vi "Requests from uServices.vi"(8 "error in (no error)":errorcluster, 9 "Data":variant, 10 "Requests":T1, 11 "Guardian in":refnum<class "Guardian.lvclass">) -> (0 "error out":errorcluster, 3 "Guardian out":refnum<class "Guardian.lvclass">)   [LabVIEW 2020, in "TALOS.lvlib" / "Guardian.lvlib" / "Guardian.lvclass"]
uses:
  Guardian.lvclass
  Guardian Messages/Broadcast to Guardians Msg/Broadcast to Guardians Msg.lvclass
  builds/Actor Framework PPL/Actor Framework.lvlibp/1abvi3w/vi.lib/ActorFramework/Actor/Actor.lvclass
  TALOS.lvlib
  Guardian Messages/Message to uService Msg/Message to uService Msg.lvclass
  C:/LabVIEW Code/TALOS/talos/Ancestor/Ancestor/Ancestor.lvclass
  C:/LabVIEW Code/TALOS/builds/Actor Framework PPL/Actor Framework.lvlibp/1abvi3w/vi.lib/ActorFramework/Actor/Actor.lvclass
  C:/LabVIEW Code/TALOS/talos/Guardian/Guardian/Guardian.lvclass
  Requests.ctl
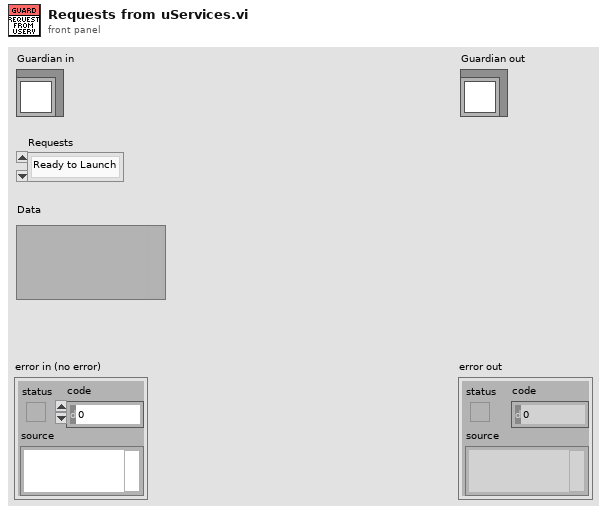
[diagram p1: front panel]
types:
  T1 = typedef "TALOS.lvlib/Guardian.lvlib/Guardian.lvclass/Requests.ctl" = enum16{"Ready to Launch", "Start RUN", "Stop RUN", "Update DAQ Params", "Update Error Listbox", "Update Run Status", "Update Kasli Log", "Run Stopped with Errors", "Switch uS View"}
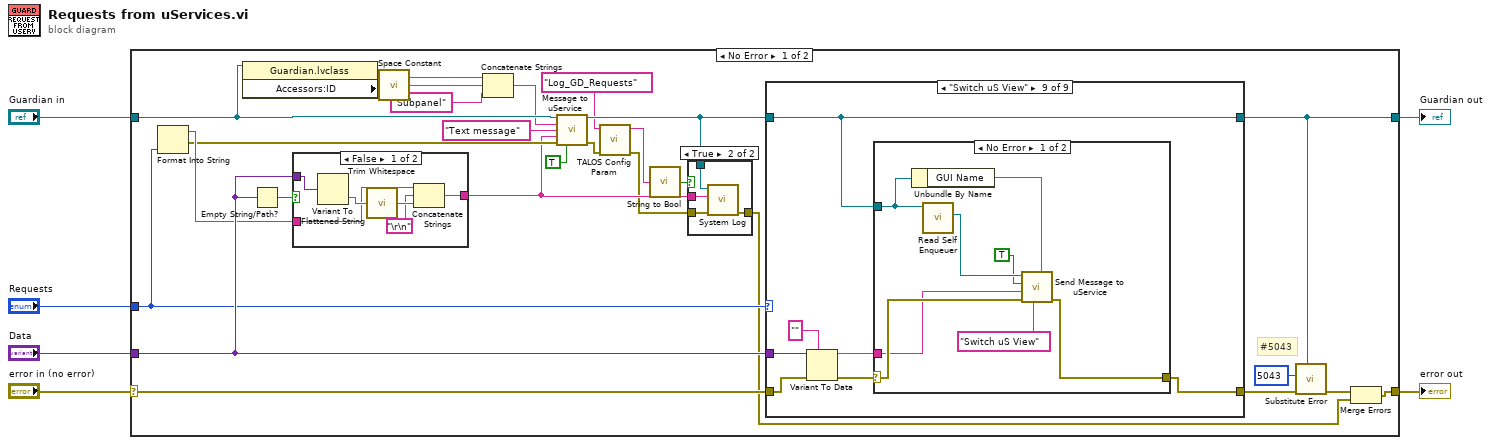
[diagram p0: block diagram]
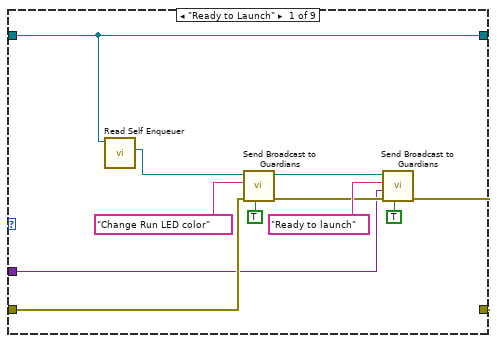
[diagram p4: hidden frame]
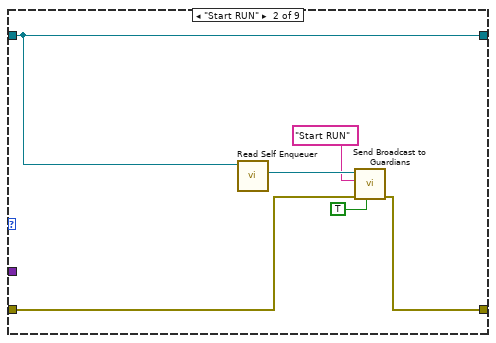
[diagram p5: hidden frame]
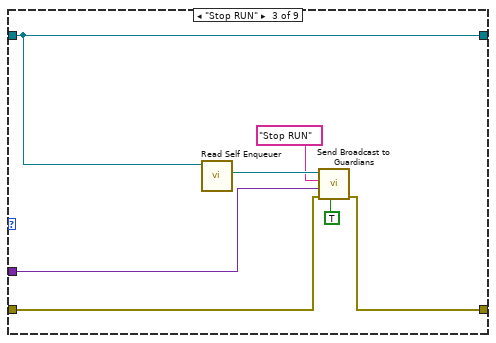
[diagram p6: hidden frame]
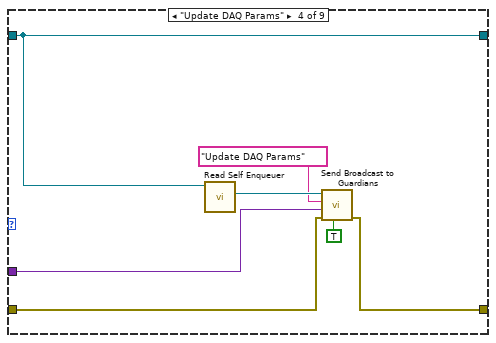
[diagram p7: hidden frame]
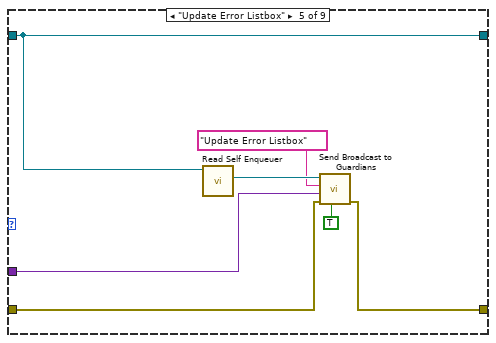
[diagram p8: hidden frame]
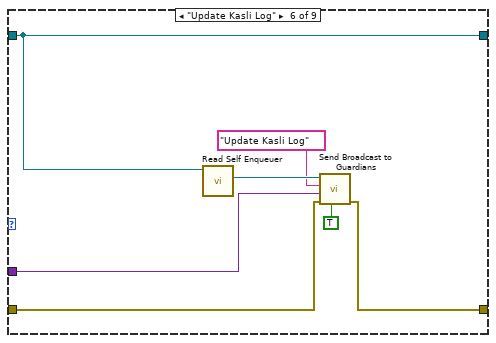
[diagram p9: hidden frame]
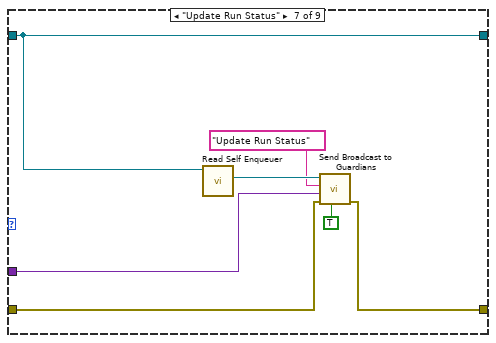
[diagram p10: hidden frame]
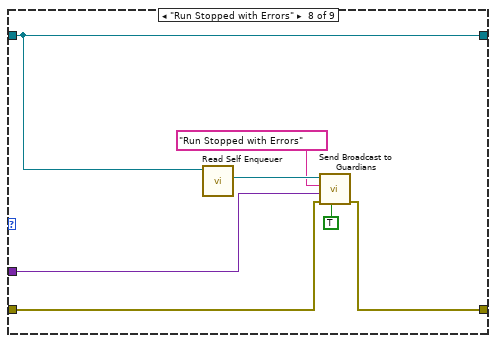
[diagram p11: hidden frame]
diagram:
  n1 = case shown="No Error" "error in (no error)" {
    selector: "error in (no error)" -> [w32 w121]
    tunnel: [w27 w121] -> w5
    tunnel: [w8 w120] -> w3
    tunnel: "Guardian in" -> [w21 w120]
    tunnel: "Requests" -> [w29 _]
    tunnel: "Data" -> [w30 _]
    frame No Error {
      # "#5043"
      n2 = Format Into String(w29) -> (resulting string=w28:string, error out=w24:errorcluster)  [unwired: 3 in]
      n3 = property class="Guardian.lvclass"(reference=w21) -> ("Accessors:ID"=w20:string)  [unwired: 1 in, 2 out]
      n4 = Empty String/Path?(string/path=w30) -> (empty?=w31:bool)
      n5 = case shown="False" w31 {
        tunnel: [w40 w44] -> w23
        tunnel: w30 -> [w39 _]
        tunnel: w28 -> [w38 w44]
        frame False {
          n6 = Variant To Flattened String(Variant=w39) -> (data string=w43:string)  [unwired: 1 out]
          n7 = call <vilib>:"Trim Whitespace.vi"("string"=w43) -> ("trimmed string"=w42:string)  [unwired: 1 in]
          n8 = Concatenate Strings(w38, "\r\n", w42) -> (w40:string)
        }
        frame True {
        }
      }
      n9 = call <vilib>:"Space Constant.vi"() -> ("String"=w17:string)
      n10 = Concatenate Strings(w20, w17, "Subpanel" ("uService ID")) -> (w19:string)
      n11 = call "Message to uService.vi"("Guardian in"=w21, "uService ID"=w19, "Message"="Text message", "Data"=w23, "error in (no error)"=w24, "Locale?"=TRUE) -> ("Guardian out"=w16:refnum<class "Guardian.lvclass">, "error out"=w11:errorcluster)  [unwired: 8 in]
      n12 = call "TALOS Config Param.vi"("error in (no error)"=w11, "Parameter Name"="Log_GD_Requests") -> ("error out"=w12:errorcluster, "Output"=w13:string)  [unwired: 8 in]
      n13 = call "String to Bool.vi"("String"=w13) -> ("Boolean"=w15:bool)
      n14 = case shown="True" w15 {
        tunnel: [w33 w37] -> w26
        tunnel: w23 -> [_ w36]
        tunnel: w16 -> [_ w35]
        tunnel: w12 -> [w33 w34]
        frame False {
        }
        frame True {
          n15 = call "System Log.vi"("error in (no error)"=w34, "Text to log"=w36, "Object in"=w35) -> ("error out"=w37:errorcluster)  [unwired: 8 in]
        }
      }
      n16 = case shown="\"Switch uS View\"" w29 {
        tunnel: w16 -> [w55 w59 w65 w73 w82 w87 w94 w101 w104]
        tunnel: [w55 w59 w65 w73 w82 w87 w94 w101 w104] -> w8
        tunnel: w32 -> [w47 w57 w68 w70 w79 w84 w91 w98 w109]
        tunnel: w30 -> [w45 _ w63 w71 w80 w85 w92 w99 w110]
        tunnel: [w53 w58 w64 w72 w81 w86 w93 w100 w105] -> w10
        frame "Ready to Launch" {
          n17 = call "Read Self Enqueuer.vi"("Actor"=w55) -> ("Self Enqueuer"=w46:refnum<class "Message Enqueuer.lvclass">)  [unwired: 10 in]
          n18 = call "Send Broadcast to Guardians.vi"("Local also?"=TRUE, "error in (no error)"=w47, "Message"="Change Run LED color", "Message Enqueuer"=w46) -> ("error out"=w48:errorcluster, "Message Enqueuer out"=w49:refnum<class "Message Enqueuer.lvclass">)  [unwired: 6 in]
          n19 = call "Send Broadcast to Guardians.vi"("Local also?"=TRUE, "error in (no error)"=w48, "Data"=w45, "Message"="Ready to launch", "Message Enqueuer"=w49) -> ("error out"=w53:errorcluster)  [unwired: 5 in, 1 out]
        }
        frame "Start RUN" {
          n20 = call "Read Self Enqueuer.vi"("Actor"=w59) -> ("Self Enqueuer"=w61:refnum<class "Message Enqueuer.lvclass">)  [unwired: 10 in]
          n21 = call "Send Broadcast to Guardians.vi"("Local also?"=TRUE, "error in (no error)"=w57, "Message"="Start RUN", "Message Enqueuer"=w61) -> ("error out"=w58:errorcluster)  [unwired: 6 in, 1 out]
        }
        frame "Stop RUN" {
          n22 = call "Read Self Enqueuer.vi"("Actor"=w65) -> ("Self Enqueuer"=w67:refnum<class "Message Enqueuer.lvclass">)  [unwired: 10 in]
          n23 = call "Send Broadcast to Guardians.vi"("Local also?"=TRUE, "error in (no error)"=w68, "Data"=w63, "Message"="Stop RUN", "Message Enqueuer"=w67) -> ("error out"=w64:errorcluster)  [unwired: 5 in, 1 out]
        }
        frame "Update DAQ Params" {
          n24 = call "Read Self Enqueuer.vi"("Actor"=w73) -> ("Self Enqueuer"=w75:refnum<class "Message Enqueuer.lvclass">)  [unwired: 10 in]
          n25 = call "Send Broadcast to Guardians.vi"("Local also?"=TRUE, "error in (no error)"=w70, "Data"=w71, "Message"="Update DAQ Params", "Message Enqueuer"=w75) -> ("error out"=w72:errorcluster)  [unwired: 5 in, 1 out]
        }
        frame "Update Error Listbox" {
          n26 = call "Read Self Enqueuer.vi"("Actor"=w82) -> ("Self Enqueuer"=w78:refnum<class "Message Enqueuer.lvclass">)  [unwired: 10 in]
          n27 = call "Send Broadcast to Guardians.vi"("Local also?"=TRUE, "error in (no error)"=w79, "Data"=w80, "Message"="Update Error Listbox", "Message Enqueuer"=w78) -> ("error out"=w81:errorcluster)  [unwired: 5 in, 1 out]
        }
        frame "Update Kasli Log" {
          n28 = call "Read Self Enqueuer.vi"("Actor"=w87) -> ("Self Enqueuer"=w89:refnum<class "Message Enqueuer.lvclass">)  [unwired: 10 in]
          n29 = call "Send Broadcast to Guardians.vi"("Local also?"=TRUE, "error in (no error)"=w84, "Data"=w85, "Message"="Update Kasli Log", "Message Enqueuer"=w89) -> ("error out"=w86:errorcluster)  [unwired: 5 in, 1 out]
        }
        frame "Update Run Status" {
          n30 = call "Read Self Enqueuer.vi"("Actor"=w94) -> ("Self Enqueuer"=w96:refnum<class "Message Enqueuer.lvclass">)  [unwired: 10 in]
          n31 = call "Send Broadcast to Guardians.vi"("Local also?"=TRUE, "error in (no error)"=w91, "Data"=w92, "Message"="Update Run Status", "Message Enqueuer"=w96) -> ("error out"=w93:errorcluster)  [unwired: 5 in, 1 out]
        }
        frame "Run Stopped with Errors" {
          n32 = call "Read Self Enqueuer.vi"("Actor"=w101) -> ("Self Enqueuer"=w103:refnum<class "Message Enqueuer.lvclass">)  [unwired: 10 in]
          n33 = call "Send Broadcast to Guardians.vi"("Local also?"=TRUE, "error in (no error)"=w98, "Data"=w99, "Message"="Run Stopped with Errors", "Message Enqueuer"=w103) -> ("error out"=w100:errorcluster)  [unwired: 5 in, 1 out]
        }
        frame "Switch uS View" {
          n34 = Variant To Data(error in=w109, type="", Variant=w110) -> (data=w106:string, error out=w107:errorcluster)
          n35 = case shown="No Error" w107 {
            selector: w107 -> [w117 w119]
            tunnel: w106 -> [w114 _]
            tunnel: [w116 w119] -> w105
            tunnel: w104 -> [w113 _]
            frame No Error {
              n36 = Unbundle By Name(w113) -> ("GUI Name"=w112:string)
              n37 = call "Read Self Enqueuer.vi"("Actor"=w113) -> ("Self Enqueuer"=w118:refnum<class "Message Enqueuer.lvclass">)  [unwired: 10 in]
              n38 = call "Send Message to uService.vi"("uService ID"=w112, "Message"="Switch uS View", "error in (no error)"=w117, "Data"=w114, "Locale?"=TRUE, "Message Enqueuer"=w118) -> ("error out"=w116:errorcluster)  [unwired: 4 in, 1 out]
            }
            frame Error {
            }
          }
        }
      }
      n39 = call "Substitute Error.vi"("LabVIEW Object"=w8, "error in (no error)"=w10, "Error Code"=5043) -> ("error out"=w9:errorcluster)  [unwired: 8 in]
      n40 = Merge Errors(w9, w26) -> (w27:errorcluster)
    }
    frame Error {
    }
  }
  "error out" <- w5
  "Guardian out" <- w3
